vi "VIH Utility - MENU - Create Menu (String).vi"(5 "comment sign ( // )":string="//", 7 "delimiter ( | )":string="|", 8 "error in":errorcluster, 10 "Menu Description":string, 11 "menu":refnum<k9>) -> (0 "error out":errorcluster, 3 "dup menu":refnum<k9>)   [LabVIEW 2014]
doc: "::: VI Helpeks :::\nCopyright (c) 2000-2026 Konstantin Shifershteyn. All rights reserved."
panel:
  # "VI Helpeks\nCopyright (c) 2012-2026 Konstantin Shifershteyn"
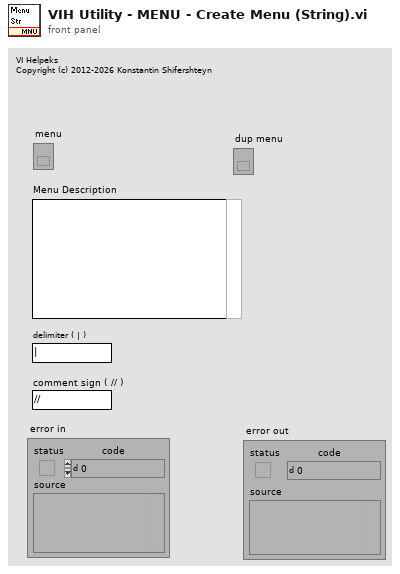
[diagram p1: front panel]
types:
  T1 = typedef "VIH Utility - MENU - Menu Item Descriptor.ctl" = cluster{"Item Name":string, "Item Tag":string, "Parent Tag":string, "Item Type":T2, "Disabled":bool, "Checked":bool}
  T2 = typedef "VIH Utility - MENU - Menu Item Type.ctl" = enum32{"Item", "SubMenu", "Separator"}
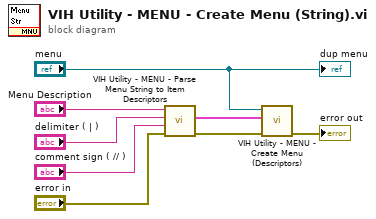
[diagram p0: block diagram]
diagram:
  n1 = call "VIH Utility - MENU - Parse Menu String to Item Descriptors.vi"("error in"="error in", "comment sign ( // )"="comment sign ( // )", "delimiter ( | )"="delimiter ( | )", "Menu Description"="Menu Description") -> ("error out"=w6:errorcluster, "Item Descriptors"=w7:T1[])  [unwired: 6 out]
  n2 = call "VIH Utility - MENU - Create Menu (Descriptors).vi"("error in"=w6, "Item Descriptors"=w7, "menu"="menu") -> ("error out"=→"error out":errorcluster)  [unwired: 8 out]
  "dup menu" <- "menu"
